vi "RemoteVI Parse Input.vi"(0 "text":string) -> (20 "kind":T1(ring), 21 "msg":u32, 22 "x":i32, 23 "y":i32, 24 "wParam":u64, 25 "lParam":i64, 26 "seq":u32, 27 "id":u64)   [LabVIEW 2020, in "RemoteVI.lvlib"]
doc: "Parses one client text message of the RemoteVI protocol: \"m msg x y wParam\" (mouse), \"k msg wParam lParam\" (key), \"a seq\" (ack) or \"x id\" (close window id, docs\\protocol.md section 7 - id not negative) or \"s id pos\" (move splitter bar id to frame coordinate pos, id not negative; id in id, pos in x) - single spaces, decimal integers with an optional leading minus, each in -2147483648..4294967295. Anything else gives kind = invalid and all numbers 0; the server ignores those. Integers wrap into the narrower output types. Pure function, cannot fail. Reference: parseInput() in tools\\lib\\protocol.mjs."
uses:
  RemoteVI.lvlib
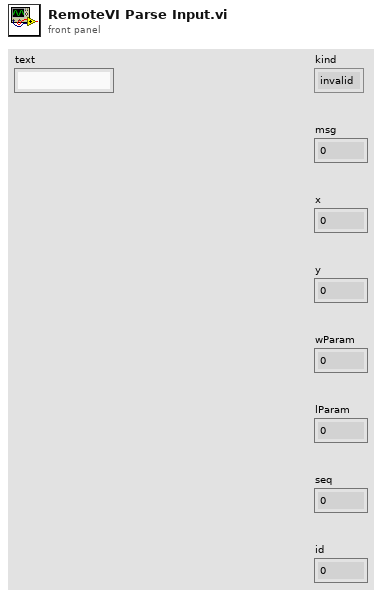
[diagram p1: front panel]
types:
  T1 = enum16{"invalid", "mouse", "key", "ack", "close", "splitter"}
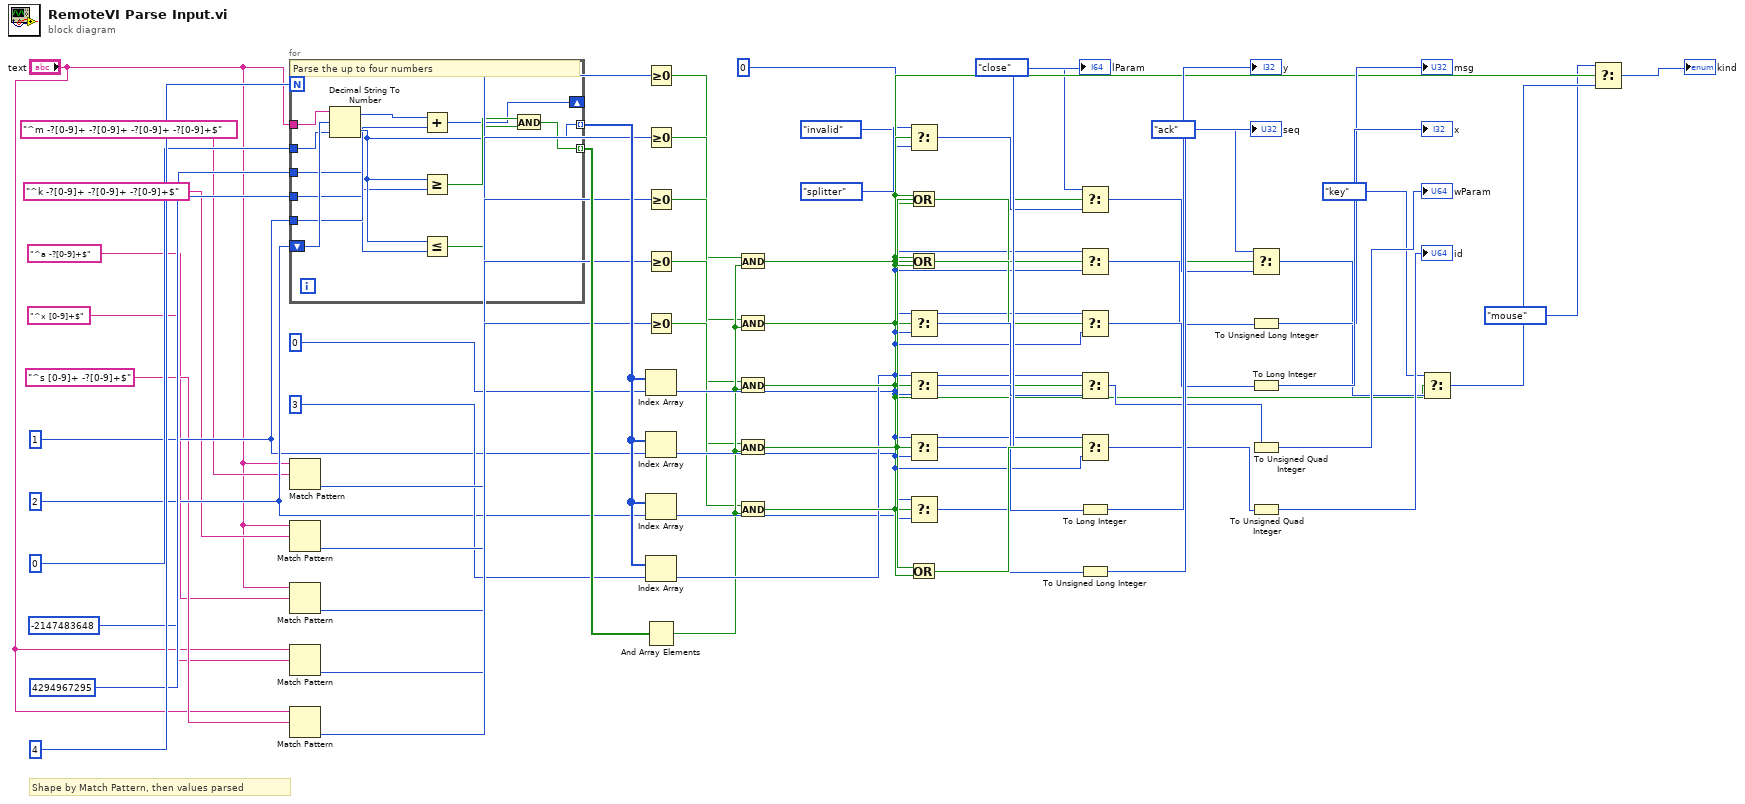
[diagram p0: block diagram]
diagram:
  w14 = i64 0
  w9 = 2
  w8 = 1
  # "Shape by Match Pattern, then values parsed"
  n1 = for {
    N: 4 -> [_]
    tunnel: "text" -> [w66]
    tunnel: i64 0 -> [w67]
    tunnel: i64 -2147483648 -> [w68]
    tunnel: i64 4294967295 -> [w69]
    tunnel: w8 -> [w70]
    shift-right: [w72] -> _
    shift-left: w9 -> [w71]
    tunnel: [w74] -> w32 mode=indexing
    tunnel: [w77] -> w33 mode=indexing
    # "Parse the up to four numbers"
    n2 = Decimal String To Number(string=w66, offset=w71, default (0L)=w67) -> (offset past number=w73:i64, number=w74:i64)
    n3 = Add(x=w73, y=w70) -> (x+y=w72:i64)
    n4 = Greater Or Equal?(x=w74, y=w68) -> (x >= y?=w75:bool)
    n5 = Less Or Equal?(x=w74, y=w69) -> (x <= y?=w76:bool)
    n6 = And(x=w75, y=w76) -> (x .and. y?=w77:bool)
  }
  n7 = Match Pattern(string="text", regular expression="^m -?[0-9]+ -?[0-9]+ -?[0-9]+ -?[0-9]+$") -> (offset past match=w21:i32)  [unwired: 1 in, 3 out]
  n8 = Match Pattern(string="text", regular expression="^k -?[0-9]+ -?[0-9]+ -?[0-9]+$") -> (offset past match=w22:i32)  [unwired: 1 in, 3 out]
  n9 = Match Pattern(string="text", regular expression="^a -?[0-9]+$") -> (offset past match=w23:i32)  [unwired: 1 in, 3 out]
  n10 = Match Pattern(string="text", regular expression="^x [0-9]+$") -> (offset past match=w24:i32)  [unwired: 1 in, 3 out]
  n11 = Match Pattern(string="text", regular expression="^s [0-9]+ -?[0-9]+$") -> (offset past match=w25:i32)  [unwired: 1 in, 3 out]
  n12 = Greater Or Equal To 0?(x=w21) -> (x >= 0?=w26:bool)
  n13 = Greater Or Equal To 0?(x=w22) -> (x >= 0?=w27:bool)
  n14 = Greater Or Equal To 0?(x=w23) -> (x >= 0?=w28:bool)
  n15 = Greater Or Equal To 0?(x=w24) -> (x >= 0?=w29:bool)
  n16 = Greater Or Equal To 0?(x=w25) -> (x >= 0?=w30:bool)
  n17 = Index Array(array=w32, index=0) -> (element=w35:i64)
  n18 = Index Array(array=w32, index=w8) -> (element=w36:i64)
  n19 = Index Array(array=w32, index=w9) -> (element=w37:i64)
  n20 = Index Array(array=w32, index=3) -> (element=w38:i64)
  n21 = And Array Elements(Boolean array=w33) -> (logical AND=w34:bool)
  n22 = And(x=w26, y=w34) -> (x .and. y?=w39:bool)
  n23 = And(x=w27, y=w34) -> (x .and. y?=w40:bool)
  n24 = And(x=w28, y=w34) -> (x .and. y?=w41:bool)
  n25 = And(x=w29, y=w34) -> (x .and. y?=w42:bool)
  n26 = And(x=w30, y=w34) -> (x .and. y?=w43:bool)
  n27 = Select(t=T1."splitter", s=w43, f=T1."invalid") -> (s? t:f=w44:T1)
  n28 = Or(x=w39, y=w40) -> (x .or. y?=w49:bool)
  n29 = Or(x=w39, y=w43) -> (x .or. y?=w51:bool)
  n30 = Select(t=w37, s=w39, f=w14) -> (s? t:f=w53:i64)
  n31 = Select(t=w36, s=w40, f=w14) -> (s? t:f=w54:i64)
  n32 = Select(t=w37, s=w40, f=w14) -> (s? t:f=→"lParam":i64)
  n33 = Select(t=w35, s=w41, f=w14) -> (s? t:f=w57:i64)
  n34 = Or(x=w42, y=w43) -> (x .or. y?=w58:bool)
  n35 = Select(t=T1."close", s=w42, f=w44) -> (s? t:f=w45:T1)
  n36 = Select(t=w35, s=w49, f=w14) -> (s? t:f=w50:i64)
  n37 = Select(t=w36, s=w51, f=w14) -> (s? t:f=w52:i64)
  n38 = Select(t=w38, s=w39, f=w54) -> (s? t:f=w55:i64)
  n39 = Select(t=w35, s=w58, f=w14) -> (s? t:f=w59:i64)
  n40 = To Long Integer(number=w53) -> (32bit integer=→"y":i32)
  n41 = To Unsigned Long Integer(number=w57) -> (unsigned 32bit integer=→"seq":u32)
  n42 = Select(t=T1."ack", s=w41, f=w45) -> (s? t:f=w46:T1)
  n43 = To Unsigned Long Integer(number=w50) -> (unsigned 32bit integer=→"msg":u32)
  n44 = To Long Integer(number=w52) -> (32bit integer=→"x":i32)
  n45 = To Unsigned Quad Integer(1:w55) -> (0:→"wParam":u64)
  n46 = To Unsigned Quad Integer(1:w59) -> (0:→"id":u64)
  n47 = Select(t=T1."key", s=w40, f=w46) -> (s? t:f=w47:T1)
  n48 = Select(t=T1."mouse", s=w39, f=w47) -> (s? t:f=→"kind":T1)
